vi "Set Datatype.vi"(8 "error in":errorcluster, 10 "Datatype":T1, 11 "Element in":refnum<class "Element.lvclass">) -> (0 "error out":errorcluster, 3 "Element out":refnum<class "Element.lvclass">)   [LabVIEW 2026, in "Element.lvclass"]
doc: "Set Datatype."
uses:
  Element.lvclass
  Type Definitions/Data types--enum.ctl
  Element.lvclass/Element.ctl
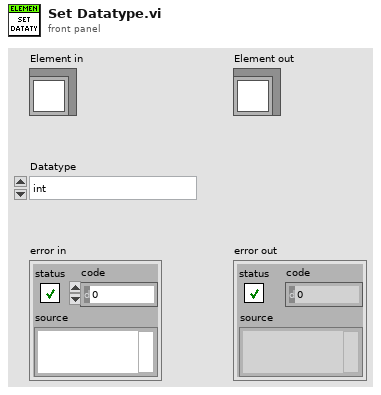
[diagram p1: front panel]
types:
  T1 = typedef "Data types--enum.ctl" = enum16{"int", "float", "bool", "str", "complex", "TypedDict", "np.bool_", "np.int8", "np.int16", "np.int32", "np.int64", "np.uint8", "np.uint16", "np.uint32", "np.uint64", "np.float32", "np.float64", "np.complex64", "np.complex128", "np.str_"}
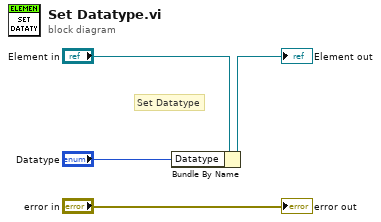
[diagram p0: block diagram]
diagram:
  # "Set Datatype"
  n1 = Bundle By Name(cluster="Element in", "Datatype"="Datatype") -> (→"Element out":refnum<class "Element.lvclass">)
  "error out" <- "error in"
